vi "Percent-Encode String.vi"(10 "String":string) -> (2 "Pct-Encoded String":string)   [LabVIEW 2013, in "openURI.lvlib"]
uses:
  openURI.lvlib
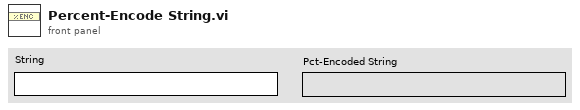
[diagram p1: front panel]
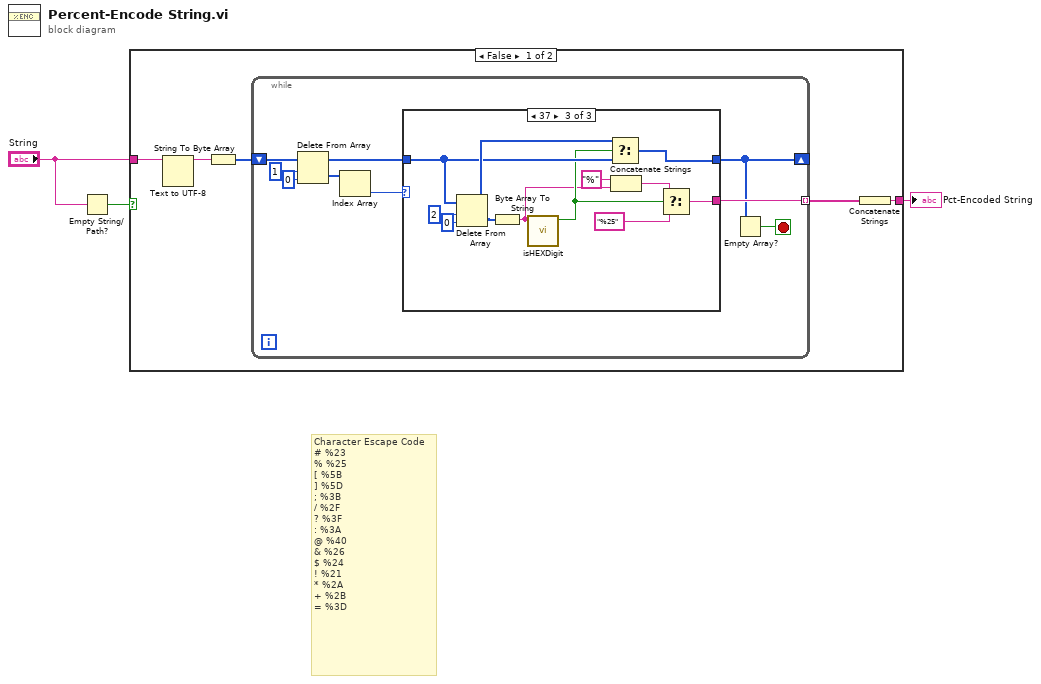
[diagram p0: block diagram]
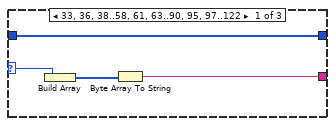
[diagram p2: hidden frame]
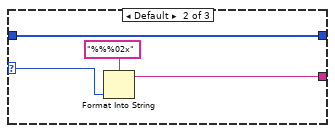
[diagram p3: hidden frame]
diagram:
  # "Character\tEscape Code\n#\t%23\n%\t%25\n[\t%5B\n]\t%5D\n;\t%3B\n/\t%2F\n?\t%3F\n:\t%3A\n@\t%40\n&\t%26\n$\t%24\n!\t%21\n*\t%2A\n+\t%2B\n=\t%3D"
  n1 = Empty String/Path?(string/path="String") -> (empty?=w2:bool)
  n2 = case shown="False" w2 {
    tunnel: "String" -> [w5 _]
    tunnel: [w6 _] -> w3
    frame False {
      n3 = Text to UTF-8(11:w5) -> (3:w4:string)  [unwired: 1 in, 1 out]
      n4 = String To Byte Array(string=w4) -> (unsigned byte array=w8:u8[])
      n5 = while {
        tunnel: [w17] -> w7 mode=indexing
        shift-right: [w10] -> _
        shift-left: w8 -> [w16]
        stop <- w9 stop-if-true
        n6 = Delete From Array(array=w16, length=1, index=0) -> (deleted portion=w13:u8[], array with subset deleted=w11:u8[])
        n7 = Index Array(array=w13) -> (element=w12:u8)  [unwired: 1 in]
        n8 = case shown="37" w12 {
          selector: w12 -> [w21 w25 _]
          tunnel: [w19 w23 w30] -> w17
          tunnel: w11 -> [w18 w22 w33]
          tunnel: [w18 w22 w32] -> w10
          frame 33, 36, 38..58, 61, 63..90, 95, 97..122 {
            n9 = Build Array(w21) -> (w20:u8[])
            n10 = Byte Array To String(unsigned byte array=w20) -> (string=w19:string)
          }
          frame Default {
            n11 = Format Into String(format string="%%%02x", w25) -> (resulting string=w23:string)  [unwired: 2 in, 1 out]
          }
          frame 37 {
            n12 = Delete From Array(array=w33, length=2, index=0) -> (deleted portion=w35:u8[], array with subset deleted=w34:u8[])
            n13 = Byte Array To String(unsigned byte array=w35) -> (string=w28:string)
            n14 = call "isHEXDigit.vi"("characters"=w28) -> ("HEX Digits"=w31:bool)  [unwired: 10 in]
            n15 = Select(t=w34, s=w31, f=w33) -> (s? t:f=w32:u8[])
            n16 = Concatenate Strings("%" ("string"), w28) -> (w27:string)
            n17 = Select(t=w27, s=w31, f="%25" ("string")) -> (s? t:f=w30:string)
          }
        }
        n18 = Empty Array?(array=w10) -> (empty?=w9:bool)
      }
      n19 = Concatenate Strings(w7) -> (w6:string)
    }
    frame True {
    }
  }
  "Pct-Encoded String" <- w3
